vi "Acquire Data.vi"(7 "user event":T2, 8 "error in":errorcluster, 9 "UI Refs":T1, 10 "Waveforms":waveform(dbl)[](array[waveform]), 11 "4way Lap":refnum<class "No Load Drift.lvclass">) -> (0 "error out":errorcluster, 3 "4way Lap out":refnum<class "No Load Drift.lvclass">)   [LabVIEW 2025, in "Flow Grind.lvlib" / "No Load Drift.lvclass"]
uses:
  No Load Drift.lvclass
  Users/Public/Documents/Sandia National Labs/TSS Plugin/CEF.lvlibp/Node/UserEventRef.ctl
  Users/Public/Documents/Sandia National Labs/TSS Plugin/Tests/XY Plotter.lvlibp/XY  Plotter/XY Plotter.lvclass
  Users/Public/Documents/Sandia National Labs/TSS Plugin/CEF.lvlibp/Node/CEF_Node.lvclass
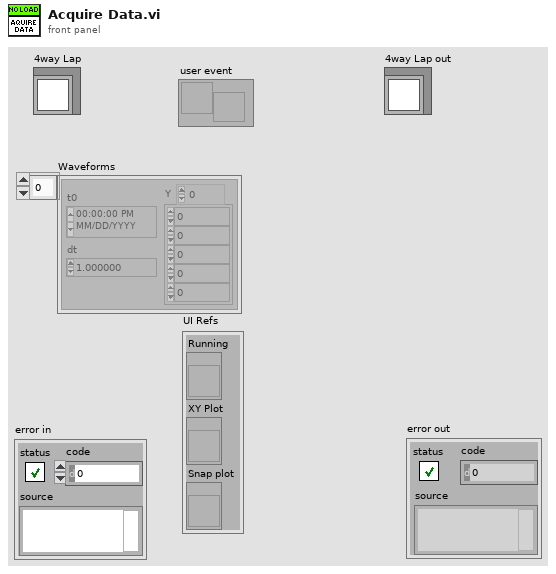
[diagram p1: front panel]
types:
  T1 = cluster{"Running":refnum<vi>, "XY Plot":refnum<vi>, "Snap plot":refnum<vi>}
  T2 = typedef "CEF.lvlibp/CEF_Node.lvclass/UserEventRef.ctl" = refnum<user-event>
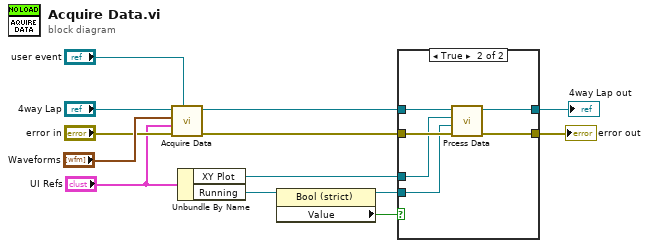
[diagram p0: block diagram]
diagram:
  n1 = call-parent "Acquire Data.vi"("user event"="user event", "error in (no error)"="error in", "UI Refs"="UI Refs", "Waveforms"="Waveforms", "XY Plotter"="4way Lap") -> ("error out"=w6:errorcluster, "XY Plotter out"=w10:refnum<class "No Load Drift.lvclass">)  [unwired: 5 in]
  n2 = Unbundle By Name("UI Refs") -> ("XY Plot"=w4:refnum<vi>, "Running"=w3:refnum<vi>)
  n3 = property class="Bool (strict)"(reference=w3) -> (reference out=w1:refnum<vi>, "Value"=w2:bool)  [unwired: 1 in, 1 out]
  n4 = case shown="True" w2 {
    tunnel: w10 -> [w15 w21]
    tunnel: [w15 w20] -> w9
    tunnel: [w14 w19] -> w8
    tunnel: w6 -> [w14 w18]
    tunnel: w4 -> [_ w17]
    tunnel: w1 -> [_ w16]
    frame False {
    }
    frame True {
      n5 = call "Prcess Data.vi"("error in (no error)"=w18, "Running"=w16, "XY Plot"=w17, "No Load"=w21) -> ("error out"=w19:errorcluster, "No Load out"=w20:refnum<class "No Load Drift.lvclass">)  [unwired: 6 in]
    }
  }
  "error out" <- w8
  "4way Lap out" <- w9
